vi "DrLL_ESR_check_ADT760.vi"(4 "Driver Name":T7, 6 "Error Code":T6, 7 "Error Query":T8, 8 "Error In":errorcluster, 11 "DriverConnect in":T1={"InterfaceType"=enum."VISA", "OpenedSession"="", "InterfaceSettings"={"Interface"=enum."RS232", "EOS 4 read"=enum."LF (\\n)", "EOS 4 write"=enum."LF (\\n)", "TMO, ms"=10000, "Sett"=variant(cluster{"Baud Rate":u32, "Data Bits":u16, "Parity":u16, "Stop Bits":u16, "Flow Control":u16, "Eho":bool} {"Baud Rate"=75, "Data Bits"=0, "Parity"=0, "Stop Bits"=0, "Flow Control"=0, "Eho"=FALSE})}}) -> (0 "Error Out":errorcluster, 3 "DriverConnect out":T1={"InterfaceType"=enum."VISA", "OpenedSession"="", "InterfaceSettings"={"Interface"=enum."RS232", "EOS 4 read"=enum."LF (\\n)", "EOS 4 write"=enum."LF (\\n)", "TMO, ms"=10000, "Sett"=variant(cluster{"Baud Rate":u32, "Data Bits":u16, "Parity":u16, "Stop Bits":u16, "Flow Control":u16, "Eho":bool} {"Baud Rate"=75, "Data Bits"=0, "Parity"=0, "Stop Bits"=0, "Flow Control"=0, "Eho"=FALSE})}})   [LabVIEW 2018]
uses:
  MOKO_LabViewLibrary/MokoLowLevel/MokoLowLovelControl/MLLC_Command.ctl
  MOKO_LabViewLibrary/MokoLowLevel/MokoLowLovelControl/MLLC_DriverName.ctl
  MOKO_LabViewLibrary/MokoLowLevel/MokoLowLovelControl/MLLC_ErrorCode.ctl
  MOKO_LabViewLibrary/MokoLowLevel/MokoLowLovelControl/MLLC_ConnectCluster.ctl
  MOKO_LabViewLibrary/MokoLowLevel/MokoLowLovelControl/MLLC_InterfaceType.ctl
  MOKO_LabViewLibrary/MokoLowLevel/MokoLowLovelControl/MLLC_OpenedSession.ctl
  MOKO_LabViewLibrary/MokoLowLevel/MokoLowLovelControl/MLLC_InterfaceSettings.ctl
  MOKO_LabViewLibrary/MokoLowLevel/MokoLowLovelControl/MLLC_InterfaceKind.ctl
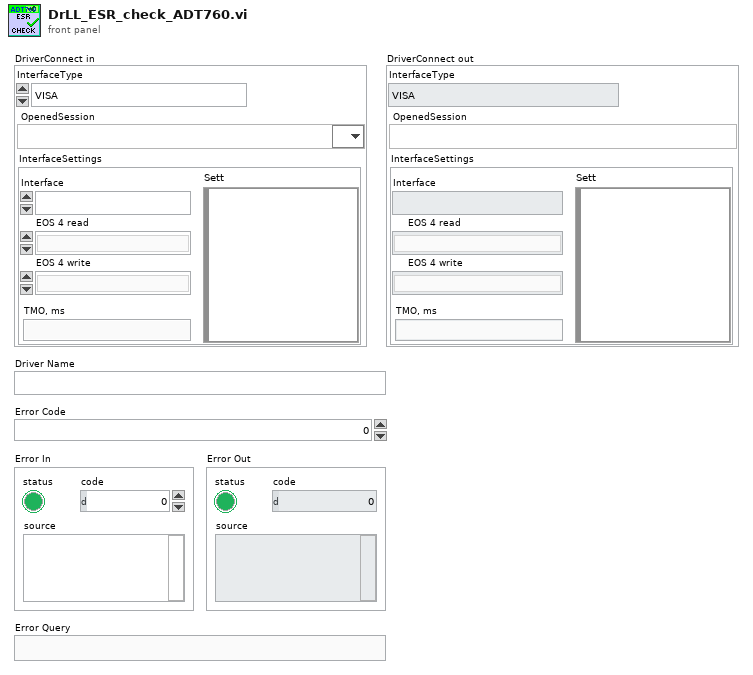
[diagram p1: front panel]
types:
  T1 = typedef "MLLC_ConnectCluster.ctl" = cluster{"InterfaceType":T2, "OpenedSession":T3, "InterfaceSettings":T4}
  T2 = typedef "MLLC_InterfaceType.ctl" = enum16{"VISA", "Prologix USB-GPIB"}
  T3 = typedef "MLLC_OpenedSession.ctl" = refnum<visa-resource-name>
  T4 = typedef "MLLC_InterfaceSettings.ctl" = cluster{"Interface":T5, "EOS 4 read":enum16{"Default (=EOS 4 write)", "CR (\\r)", "LF (\\n)", "None"}, "EOS 4 write":enum16{"CR+LF (\\r\\n)", "CR (\\r)", "LF (\\n)", "None"}, "TMO, ms":i32, "Sett":variant}
  T5 = typedef "MLLC_InterfaceKind.ctl" = enum16{"RS232", "GPIB", "USB", "Ethernet", "another"}
  T6 = typedef "MLLC_ErrorCode.ctl" = u32
  T7 = typedef "MLLC_DriverName.ctl" = string
  T8 = typedef "MLLC_Command.ctl" = string
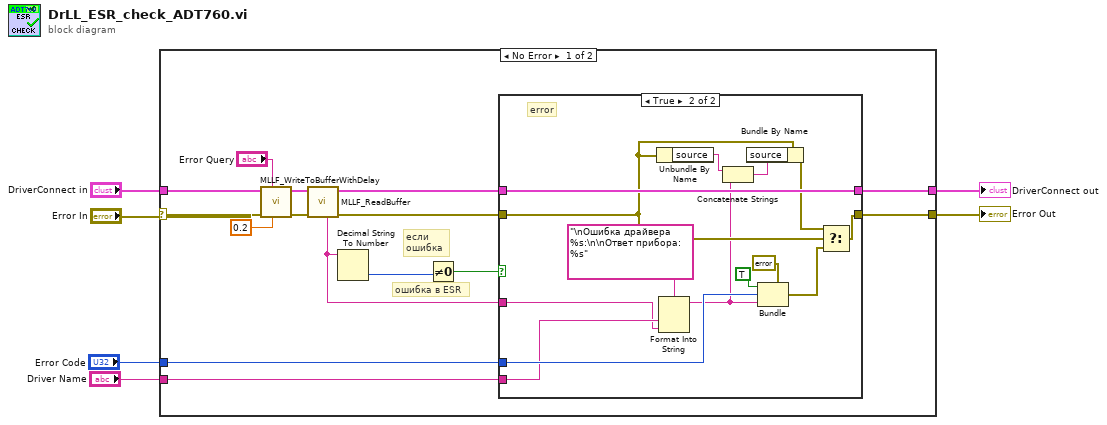
[diagram p0: block diagram]
diagram:
  n1 = case shown="No Error" "Error In" {
    selector: "Error In" -> [w20 w39]
    tunnel: [w21 w39] -> w3
    tunnel: [w19 w38] -> w1
    tunnel: "Error Code" -> [w18 _]
    tunnel: "Driver Name" -> [w17 _]
    tunnel: "DriverConnect in" -> [w7 w38]
    frame No Error {
      # "ошибка в ESR"
      # "если \nошибка"
      n2 = call "MLLF_WriteToBufferWithDelay.vi"("Delay Time ( 0,05 s)"=0.2 ("Delay Time (s)"), "Command"="Error Query", "Error In"=w20, "DriverConnect in"=w7) -> ("Error Out"=w16:errorcluster, "DriverConnect out"=w15:T1)  [unwired: 6 in]
      n3 = call "MLLF_ReadBuffer.vi"("Error In"=w16, "DriverConnect in"=w15) -> ("Error Out"=w12:errorcluster, "DriverConnect out"=w13:T1, "String"=w10:string)  [unwired: 6 in]
      n4 = Decimal String To Number(string=w10) -> (number=w14:i32)  [unwired: 2 in, 1 out]
      n5 = Not Equal To 0?(x=w14) -> (x != 0?=w11:bool)
      n6 = case shown="True" w11 {
        tunnel: w13 -> [w23 w32]
        tunnel: [w23 w32] -> w19
        tunnel: [w22 w25] -> w21
        tunnel: w12 -> [w22 w31]
        tunnel: w18 -> [_ w34]
        tunnel: w17 -> [_ w33]
        tunnel: w10 -> [_ w24]
        frame False {
          # "no error"
        }
        frame True {
          # "error"
          n7 = Unbundle By Name(w31) -> ("source"=w30:string)
          n8 = Format Into String(format string="\nОшибка драйвера %s:\n\nОтвет прибора: %s", w33, w24) -> (resulting string=w28:string)  [unwired: 2 in, 1 out]
          n9 = Concatenate Strings(w30, w28) -> (w29:string)
          n10 = Bundle By Name(cluster=w31, "source"=w29) -> (w27:errorcluster)
          n11 = Bundle(cluster=errorcluster {"status"=FALSE, "code"=0, "source"=""} ("error out"), "status"=TRUE ("Status"), "code"=w34, "source"=w28) -> (w26:errorcluster)
          n12 = Select(t=w27, s=w31, f=w26) -> (s? t:f=w25:errorcluster)
        }
      }
    }
    frame Error {
    }
  }
  "Error Out" <- w3
  "DriverConnect out" <- w1
